vi "WIFI_CON.vi"(8 "error in":errorcluster) -> (0 "error out":errorcluster, 1 "Command Response":string, 2 "Result":string, 3 "RESULT":bool)   [LabVIEW 2021]
uses:
  10054_Control Folder/Support/Relay_no.ctl
  DUT/DUT_Cmd.ctl
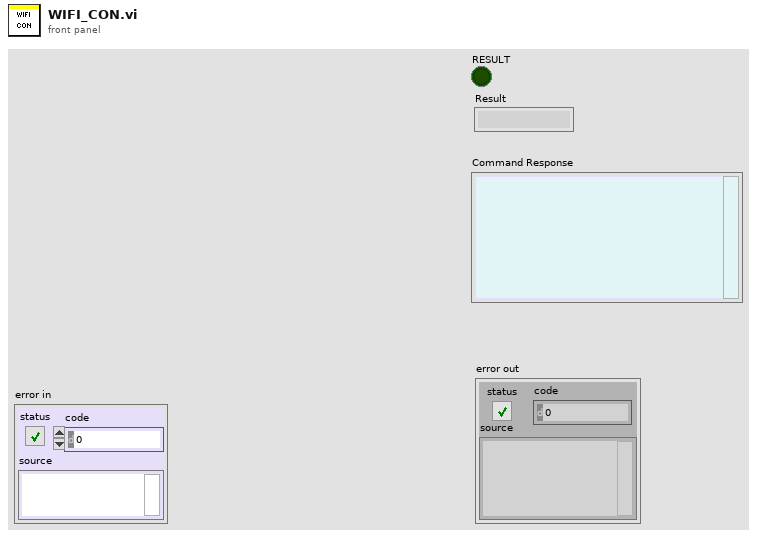
[diagram p1: front panel]
types:
  T1 = typedef "Relay_no.ctl" = enum16{"Init", "write&Read", "PCB Serial Write & Read", "PCB Write SSD & Password", "Read Wifi state", "Reset", "Close"}
  T2 = typedef "DUT_Cmd.ctl" = enum16{"Unlock serial", "Stop console logs", "Release emergency at start", "Read firmware", "WiFi credentials", "WiFi connected", "WiFi SSID", "Board revision", "ADC_NTC_TEMP", "ADC_TYPE2_RCD_CURRENT", "PCBA serial write", "PCBA serial readback", "Start energy meter", "Energy meter Vac", "Energy meter Iac", "Energy meter PF", "Energy meter energy", "Provision", "Set gateway identity", "CP checklist", "Earth detect", "D+M sense unplugged", "D+M sense plugged", "Output relay weld", "Start diagnostics", "Relay 1 on", "Relay 2 on", "Emergency pressed", "Release emergency", "Emergency released", "Unlock serial for 5 A", "Board current (5 A)", "Unlock serial for 15 A", "Board current (15 A)", "Unlock serial for 0 A", "NFC tag", "Start diagnostics again", "Relay 2 off", "Relay 1 off", "End diagnostics", "Load current (5 A) [No USB station]", "Load current (15 A) [No USB station]", "Load current (0 A) [No USB station]", "NFC tag [No USB station]", "Battery Voltage", "FW Power reset", "Notification LED", "O/P Relay weld Detection", "Earth Detection", "12V ", "5V", "3.3V", "Reboot"}
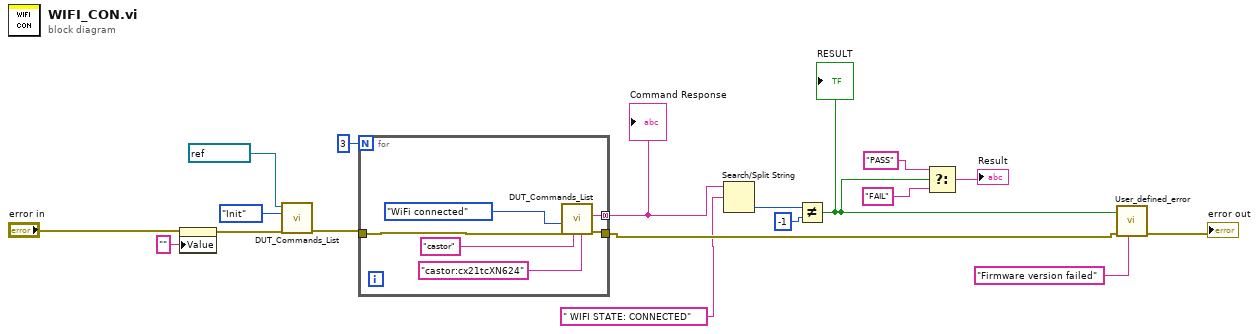
[diagram p0: block diagram]
diagram:
  n1 = property on="Command Response" class="Str"(error in="error in", "Value"="" ("Command Response")) -> (error out=w6:errorcluster)  [unwired: 1 in, 1 out]
  n2 = call "DUT_Commands_List.vi"("error in"=w6, "Operation"=Relay_no."Init", "Resource In"=refnum<visa-resource-name> "COM3") -> ("error out"=w5:errorcluster)  [unwired: 6 in, 2 out]
  n3 = for {
    N: 3 -> [_]
    tunnel: [w24] -> w10 mode=concatenating
    tunnel: w5 -> [w20]
    tunnel: [w21] -> w8
    n4 = call "DUT_Commands_List.vi"("Password"="castor:cx21tcXN624", "SSID"="castor", "error in"=w20, "DUT Cmd"=DUT_Cmd."WiFi connected") -> ("error out"=w21:errorcluster, "Command Response"=w24:string)  [unwired: 5 in, 1 out]
  }
  "Command Response" <- w10
  n5 = Search/Split String(string=w10, search string/char (-)=" WIFI STATE: CONNECTED") -> (offset of match=w17:i32)  [unwired: 1 in, 2 out]
  n6 = Not Equal?(x=w17, y=-1) -> (x != y?=w14:bool)
  "RESULT" <- w14
  n7 = Select(t="PASS", s=w14, f="FAIL") -> (s? t:f=→"Result":string)
  n8 = call "User_defined_error.vi"("Error Msg"="Firmware version failed" ("source"), "error in"=w8, "Result"=w14) -> ("error Out"=→"error out":errorcluster)  [unwired: 8 in]
